vi "Add Error Core.vi"(8 "error in (no error)":errorcluster, 10 "String to Append":string, 11 "Error":T1) -> (0 "error out":errorcluster)   [LabVIEW 2021, in "XNET CAN RW.lvclass"]
uses:
  XNET CAN RW.lvclass
  typedef/Errors.ctl
  XNET CAN RW.lvclass/XNET CAN RW.ctl
  <vilib>/CIF Foundation/CIF Utilities/Errors/Errors_CIF_U.lvlib
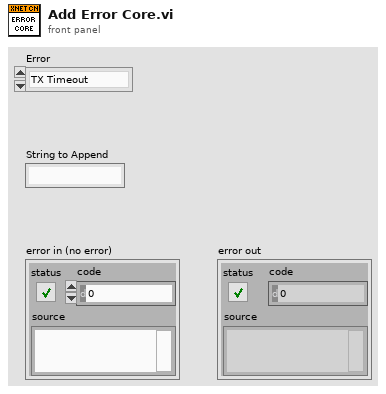
[diagram p1: front panel]
types:
  T1 = typedef "XNET CAN RW.lvclass/Errors.ctl" = enum16{"TX Timeout", "Packet Length", "Invalid Start Time", "Bus Fault"}
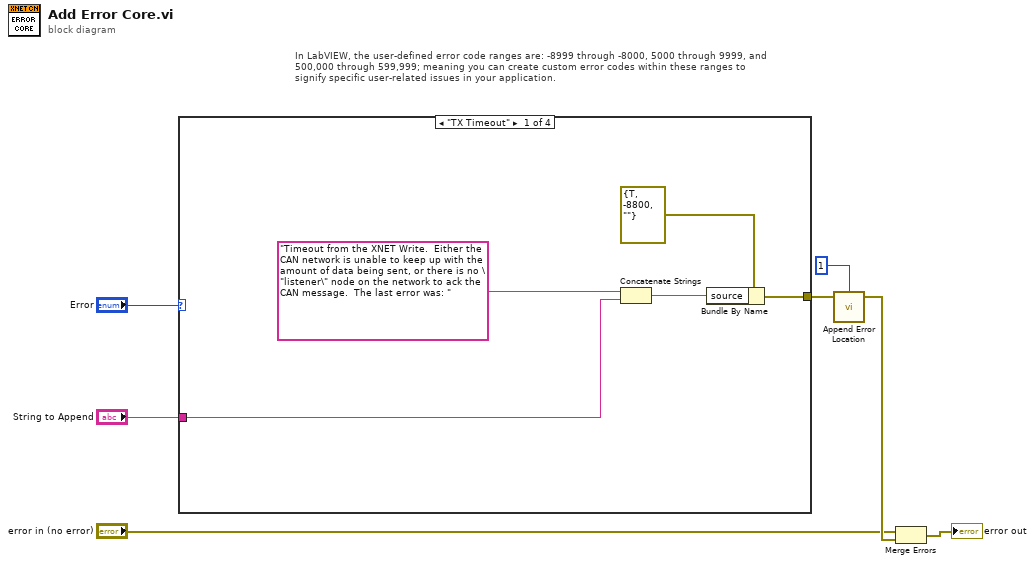
[diagram p0: block diagram]
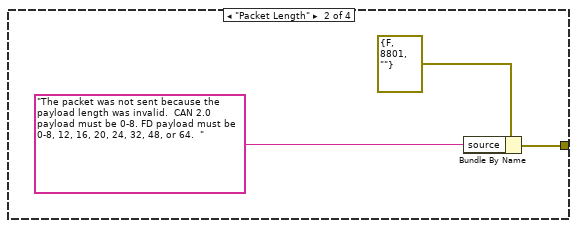
[diagram p2: hidden frame]
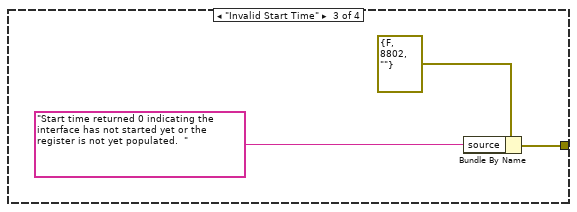
[diagram p3: hidden frame]
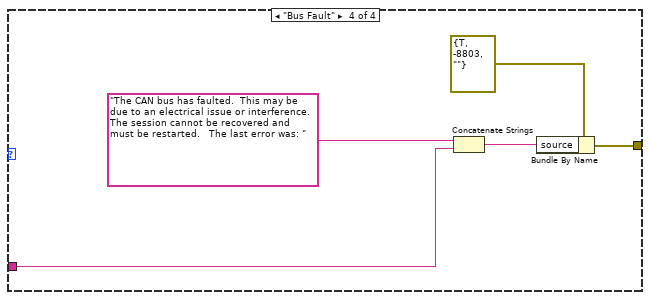
[diagram p4: hidden frame]
diagram:
  # "In LabVIEW, the user-defined error code ranges are: -8999 through -8000, 5000 through 9999, and 500,000 through 599,999; meaning you can create custom error codes within these ranges to signify specific user-related issues in your application."
  n1 = case shown="\"TX Timeout\"" "Error" {
    tunnel: "String to Append" -> [w8 _ _ w19]
    tunnel: [w11 w14 w17 w22] -> w6
    frame "TX Timeout" {
      n2 = Concatenate Strings("Timeout from the XNET Write.  Either the CAN network is unable to keep up with the amount of data being sent, or there is no \"listener\" node on the network to ack the CAN message.  The last error was: " ("source"), w8) -> (w9:string)
      n3 = Bundle By Name(cluster=errorcluster {"status"=TRUE, "code"=-8800, "source"=""} ("Invalid ID"), "source"=w9) -> (w11:errorcluster)
    }
    frame "Packet Length" {
      n4 = Bundle By Name(cluster=errorcluster {"status"=FALSE, "code"=8801, "source"=""} ("Invalid ID"), "source"="The packet was not sent because the payload length was invalid.  CAN 2.0 payload must be 0-8. FD payload must be 0-8, 12, 16, 20, 24, 32, 48, or 64.  ") -> (w14:errorcluster)
    }
    frame "Invalid Start Time" {
      n5 = Bundle By Name(cluster=errorcluster {"status"=FALSE, "code"=8802, "source"=""} ("Invalid ID"), "source"="Start time returned 0 indicating the interface has not started yet or the register is not yet populated.  ") -> (w17:errorcluster)
    }
    frame "Bus Fault" {
      n6 = Concatenate Strings("The CAN bus has faulted.  This may be due to an electrical issue or interference.  The session cannot be recovered and must be restarted.   The last error was: " ("source"), w19) -> (w20:string)
      n7 = Bundle By Name(cluster=errorcluster {"status"=TRUE, "code"=-8803, "source"=""} ("Invalid ID"), "source"=w20) -> (w22:errorcluster)
    }
  }
  n8 = call <vilib>:"Append Error Location.vi"("error in (no error)"=w6, "Chain Depth"=1) -> ("error out"=w7:errorcluster)  [unwired: 3 in]
  n9 = Merge Errors("error in (no error)", w7) -> (→"error out":errorcluster)
